vi "shutdown.vi"(8 "error in":errorcluster, 11 "Target Runtime in":refnum<class "PL_Target Runtime.lvclass">) -> (0 "error out":errorcluster)   [LabVIEW 2013, in "PL_Target Runtime.lvclass"]
doc: "Performs any shutdown operations necessary to close any references initialized by the target. This should be called last after shutting down all engines and modules used by the target."
uses:
  PL_Target Runtime.lvclass
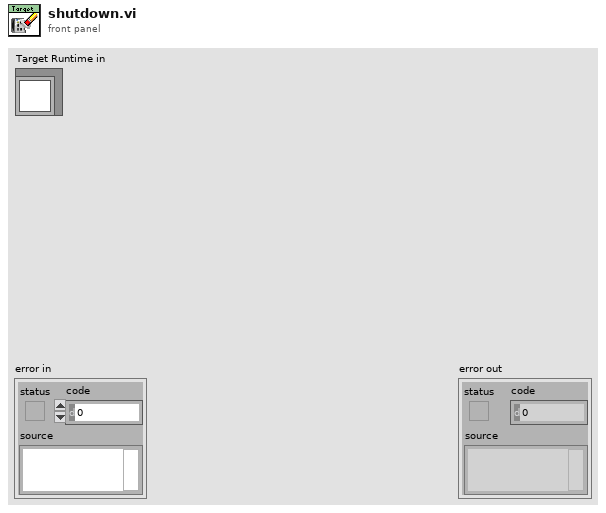
[diagram p1: front panel]
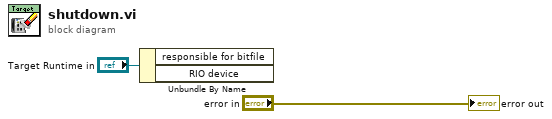
[diagram p0: block diagram]
diagram:
  n1 = Unbundle By Name("Target Runtime in") -> ()  [unwired: 2 out]
  "error out" <- "error in"
